vi "SMTP Email Command.vi"(4 "error in (no error)":errorcluster caption="entrée d'erreur (pas d'erreur)", 6 "command":string caption="commande", 7 "smtp session":T1 caption="session smtp") -> (0 "error out":errorcluster caption="sortie d'erreur", 1 "reply":string caption="réponse", 2 "reply code":i32 caption="code de réponse", 3 "smtp session out":T1 caption="session smtp en sortie")   [LabVIEW 2022 SP3, in "Copie de NI_SMTPEmail.lvlib"]
doc: "VI polyvalent qui envoie n'importe quel type de message (commande) au serveur SMTP en utilisant \"Session SMTP\", et qui reçoit une chaîne de réponse (qui peut avoir plusieurs lignes conformément à la norme RFC821)."
uses:
  Copie de NI_SMTPEmail.lvlib
  SMTP Email Session.ctl
panel:
  in  "tcp connection":refnum<k5> caption="connexion tcp"
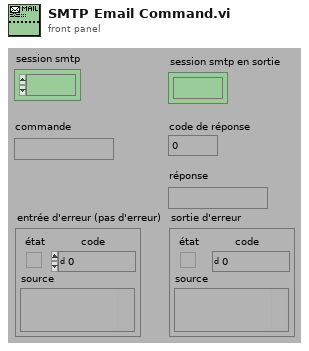
[diagram p1: front panel]
types:
  T1 = typedef "Copie de NI_SMTPEmail.lvlib/SMTP Email Session.ctl" = refnum<k1>
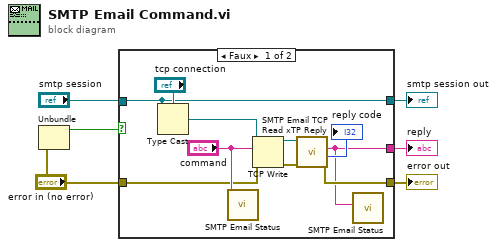
[diagram p0: block diagram]
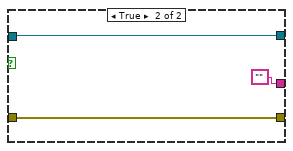
[diagram p2: hidden frame]
diagram:
  n1 = Unbundle("error in (no error)") -> ("status"=w2:bool)  [unwired: 2 out]
  n2 = case shown="Faux" w2 {
    tunnel: "smtp session" -> [w11 w19]
    tunnel: [w14 w17] -> w1
    tunnel: [w9 ""] -> w5
    tunnel: [w11 w19] -> w4
    tunnel: "error in (no error)" -> [w7 w17]
    frame False {
      n3 = Type Cast(type="tcp connection", x=w11) -> (*(type *) &x=w12:refnum<k5>)
      n4 = call "SMTP Email Status"("action string"="command") -> ()  [unwired: 9 in, 2 out]
      n5 = TCP Write(connection ID=w12, data in="command", error in (no error)=w7) -> (connection ID out=w15:refnum<k5>, error out=w16:errorcluster)  [unwired: 1 in, 1 out]
      n6 = call "SMTP Email TCP Read xTP Reply.vi"("error in (no error)"=w16, "buffered tcp connection"=w15) -> ("error out"=w14:errorcluster, "reply code"=→"reply code":i32, "reply string"=w9:string)  [unwired: 6 in, 1 out]
      n7 = call "SMTP Email Status"("status string"=w9) -> ()  [unwired: 9 in, 2 out]
    }
    frame True {
    }
  }
  "error out" <- w1
  "reply" <- w5
  "smtp session out" <- w4
